vi "Global-test.vi"() -> ()   [LabVIEW 2020, in "Sgraph_lib_V1.lvlib"]
uses:
  Builds/Sgraph_lib_V1.lvlib
panel:
  in  "File":string
  out "Boolean":bool
  in  "String":string
  in  "Test":dbl
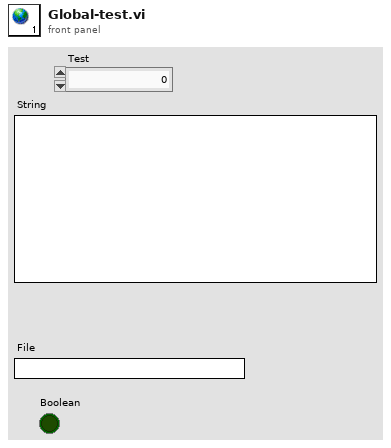
[diagram p1: front panel]
diagram:
